vi "Capture_Process_Sample.vi"(8 "error in (no error)":errorcluster={"status"=FALSE, "code"=0, "source"="\"\""}, 10 "timestamped ParameterSnapshot":string, 11 "Session ID":string) -> (0 "error out":errorcluster={"status"=FALSE, "code"=0, "source"="\"\""}, 2 "status ok":bool, 3 "Updated accumulator":string)   [LabVIEW 2026]
doc: "INTENT: Update selected sample accumulators. LOGIC: Count valid samples; compute sum/min/max, optional raw sample buffering with gaps and quality flags."
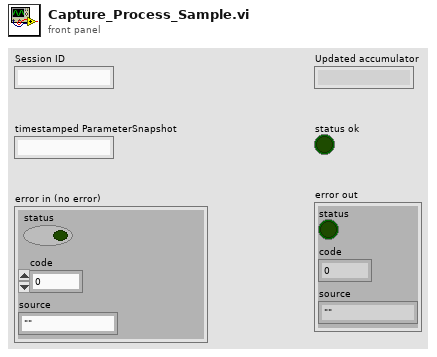
[diagram p1: front panel]
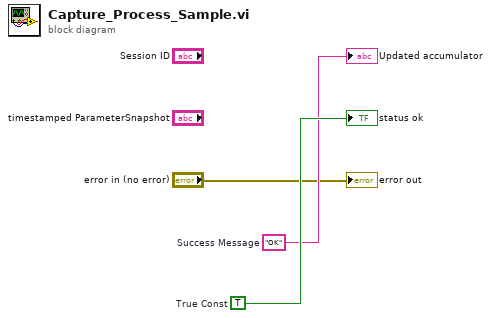
[diagram p0: block diagram]
diagram:
  w3 = TRUE  # True Const
  w2 = "OK"  # Success Message
  "Updated accumulator" <- w2
  "status ok" <- w3
  "error out" <- "error in (no error)"
